vi "_LabeledRectangleDrawBoundingBox.vi"(7 "GroupName":string, 8 "error in":errorcluster, 9 "Color":u32(colorbox)=16711680, 10 "BoundingBox":T1, 11 "Image Reference In":T3) -> (0 "error out":errorcluster, 3 "Image Reference Out":T3)   [LabVIEW 2020, in "OpenLvVision_Overlays.lvlib"]
uses:
  <vilib>/OpenLvVision/OpenLvVision_Image/Management/TypeDef/OLV Image.ctl
  OpenLvVision_Overlays.lvlib
  TypeDefs/DrawingMode.ctl
  <vilib>/OpenLvVision/OpenLvVision_Image/Management/OLV Management.lvlib
  TypeDefs/PointI32.ctl
  TypeDefs/RotatedRectangle.ctl
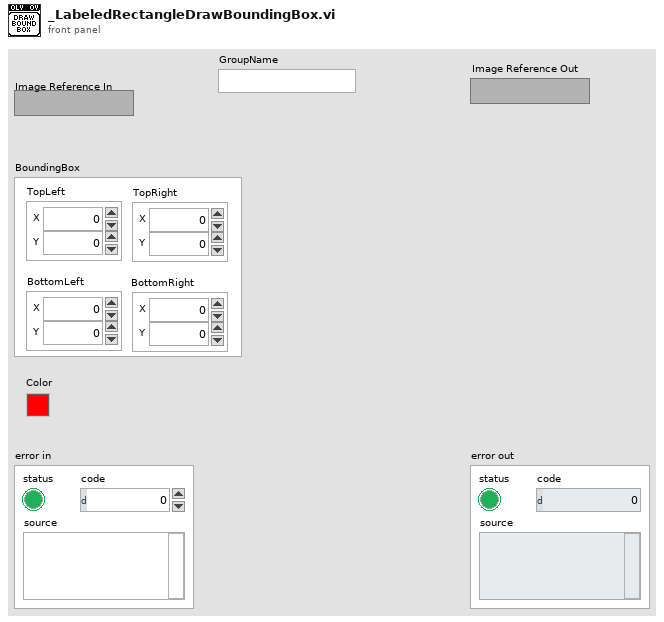
[diagram p1: front panel]
types:
  T1 = typedef "OpenLvVision_Overlays.lvlib/RotatedRectangle.ctl" = cluster{"TopLeft":T2, "TopRight":T2, "BottomRight":T2, "BottomLeft":T2}
  T2 = typedef "OpenLvVision_Overlays.lvlib/PointI32.ctl" = cluster{"X":i32, "Y":i32}
  T3 = typedef "OLV OpenLvVision_Image.lvlib/OLV Management.lvlib/OLV Image.ctl" = refnum<image>
  T4 = typedef "OpenLvVision_Overlays.lvlib/DrawingMode.ctl" = enum16{"Frame", "Fill"}
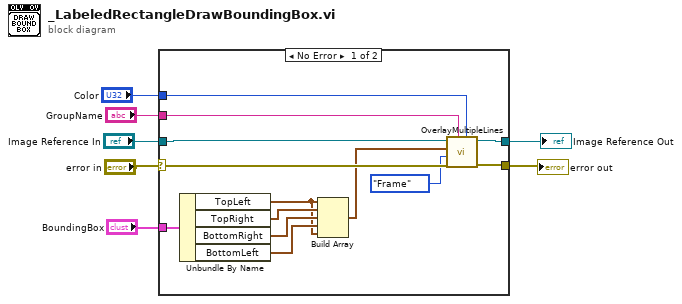
[diagram p0: block diagram]
diagram:
  n1 = case shown="No Error" "error in" {
    selector: "error in" -> [w17 w21]
    tunnel: [w19 w21] -> w6
    tunnel: "Image Reference In" -> [w18 w22]
    tunnel: [w20 w22] -> w5
    tunnel: "GroupName" -> [w16 _]
    tunnel: "Color" -> [w15 _]
    tunnel: "BoundingBox" -> [w13 _]
    frame No Error {
      n2 = Unbundle By Name(w13) -> ("TopLeft"=w9:T2, "TopRight"=w12:T2, "BottomRight"=w11:T2, "BottomLeft"=w10:T2)
      n3 = Build Array(w9, w12, w11, w10, w9) -> (w8:T2[])
      n4 = call "OverlayMultipleLines.vi"("Color"=w15, "GroupName"=w16, "error in"=w17, "Drawing Mode (Frame)"=DrawingMode."Frame", "Points"=w8, "Image Reference In"=w18) -> ("error out"=w19:errorcluster, "Image Reference Out"=w20:T3)  [unwired: 4 in]
    }
    frame Error {
    }
  }
  "error out" <- w6
  "Image Reference Out" <- w5
